vi "FACTORIAL SUB VI.vi"(11 "N":i32) -> (3 "x*y":i32)   [LabVIEW 2018]
panel:
  # "nCr= n!/(n-r)!"
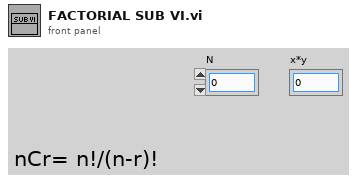
[diagram p1: front panel]
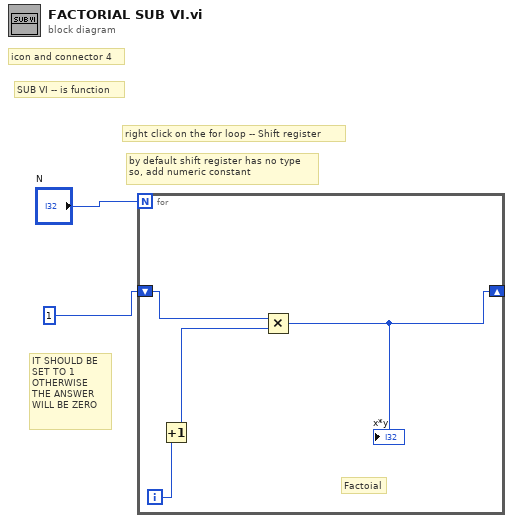
[diagram p0: block diagram]
diagram:
  # "by default shift register has no type \nso, add numeric constant"
  # "IT SHOULD BE \nSET TO 1\nOTHERWISE\nTHE ANSWER \nWILL BE ZERO"
  # "right click on the for loop -- Shift register"
  # "icon and connector 4"
  # "SUB VI -- is function"
  n1 = for {
    N: "N" -> [_]
    shift-right: [w4] -> _
    shift-left: 1 -> [w6]
    i -> [w5]
    # "Factoial"
    n2 = Increment(x=w5) -> (x+1=w3:i32)
    n3 = Multiply(x=w6, y=w3) -> (x*y=w4:i32)
    "x*y" <- w4
  }
